vi "ClassProvidor_GoopOptionsDialog.vi"(8 "error in (no error)":errorcluster) -> (0 "error out":errorcluster)   [LabVIEW 2020]
uses:
  Provider_EndevoGOOP300/EndevoProviderName.ctl
  Provider_EndevoGOOP400/EndevoG4ProviderName.ctl
panel:
  out "ProductPicture":picture
  in  "_InstallNewClassProvider":bool
  in  "_RemoveClassProvider":bool
  in  "_HelpGoopOption":bool
  in  "_AddClassProvider":bool
  out "Tab":enum32{"Select", "Add"}(tab)
  in  "ModifyProviders":bool
  in  "_CurrentClassProvider":u16(ring) caption="Current Class provider to use:" items=["LVClass by value", "By Reference (GOOP3)", "By Reference DVR (GOOP4)"]
  in  "_ConfigureCurrentClassProvider":bool
  in  "_ProviderClassReaderPath":path caption="Provider Class Reader Path"
  in  "_ProviderClassWriterPath":path caption="Provider Class Writer Path"
  in  "_ProviderName":string caption="ProviderName"
  in  "Cancel":bool
  in  "OK":bool
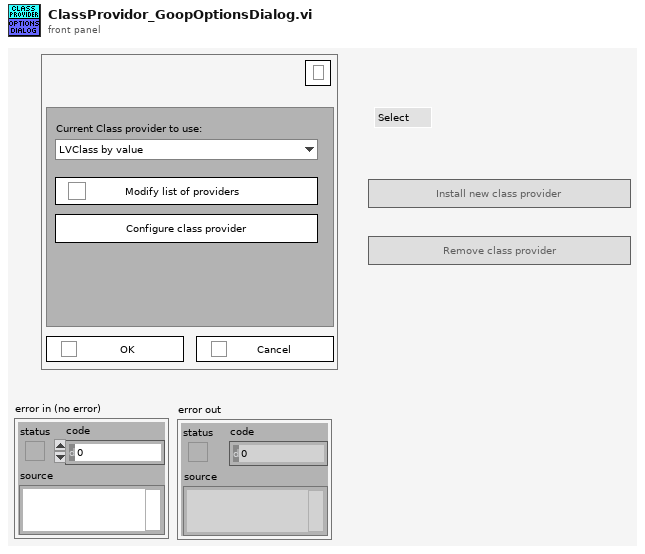
[diagram p1: front panel]
types:
  T1 = cluster{"ClassProviders":string[], "Path":path, "ClassConfig":path, "ClassProviders(Translated)":string[]}
  T2 = typedef "EndevoG4ProviderName.ctl" = enum16{"EndevoGOOP400"}
  T3 = typedef "EndevoProviderName.ctl" = enum16{"EndevoGOOP300"}
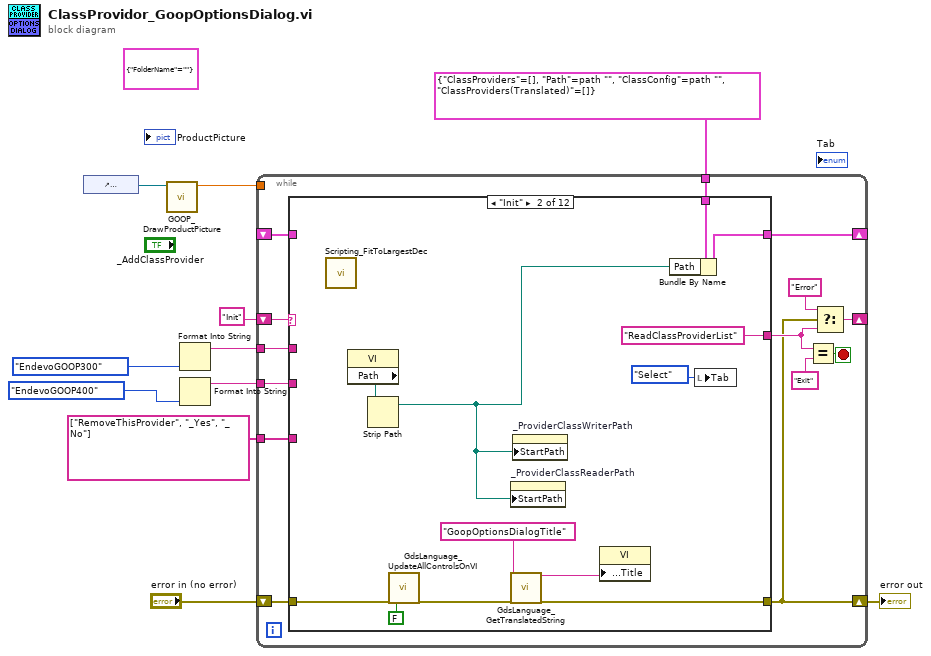
[diagram p0: block diagram]
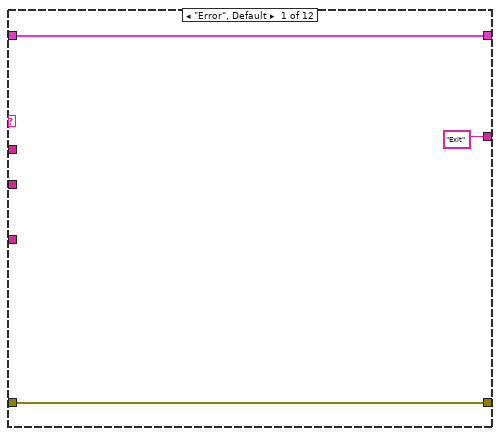
[diagram p2: hidden frame]
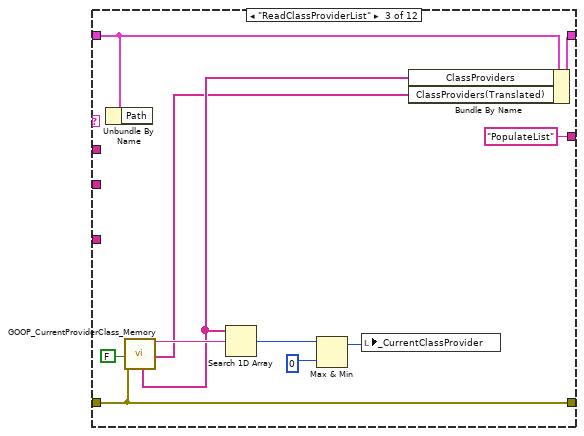
[diagram p3: hidden frame]
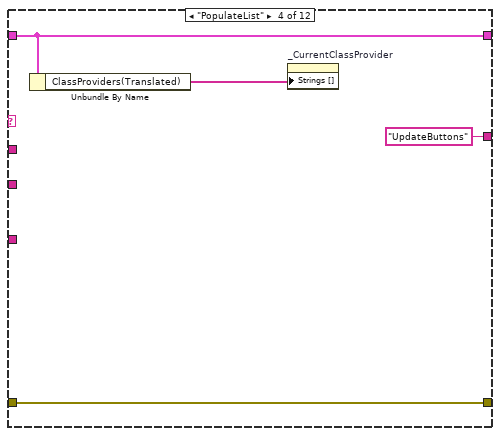
[diagram p4: hidden frame]
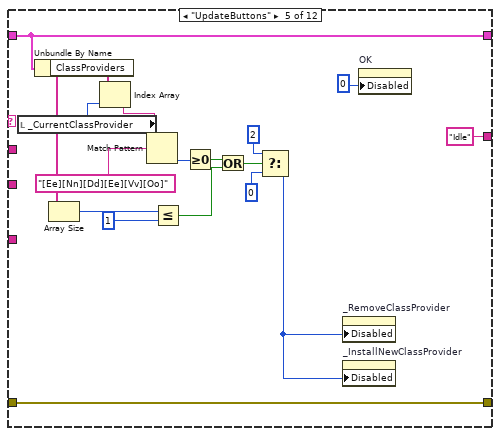
[diagram p5: hidden frame]
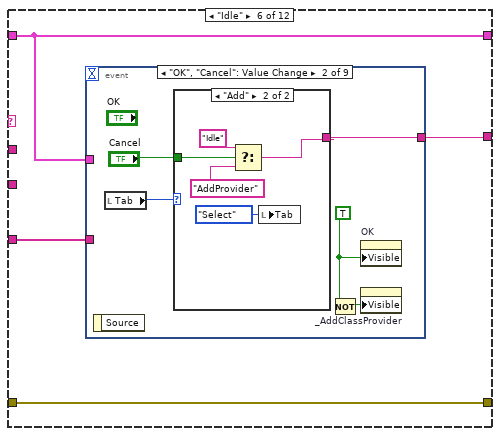
[diagram p6: hidden frame]
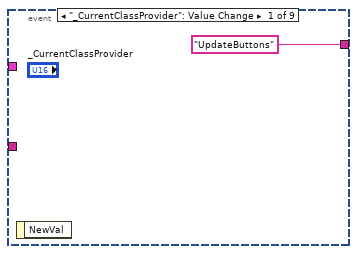
[diagram p7: hidden frame]
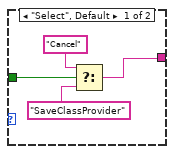
[diagram p8: hidden frame]
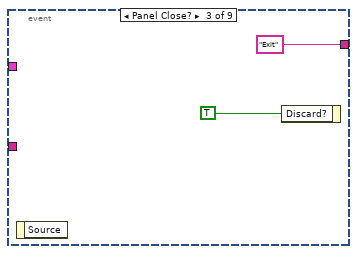
[diagram p9: hidden frame]
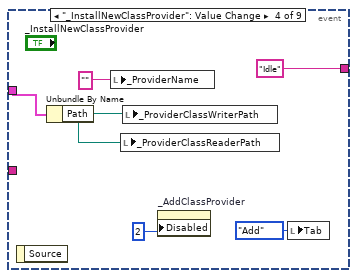
[diagram p10: hidden frame]
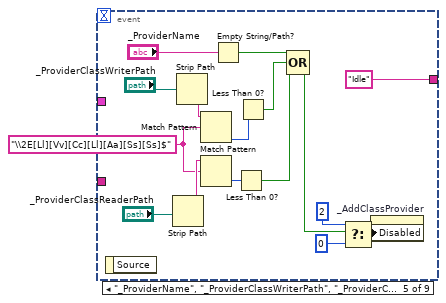
[diagram p11: hidden frame]
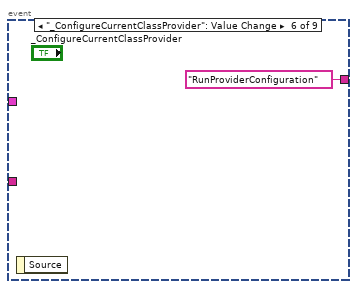
[diagram p12: hidden frame]
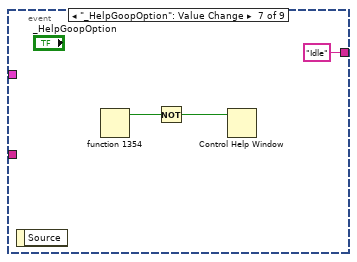
[diagram p13: hidden frame]
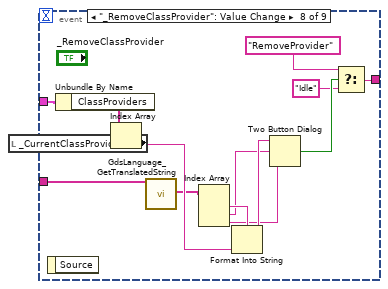
[diagram p14: hidden frame]
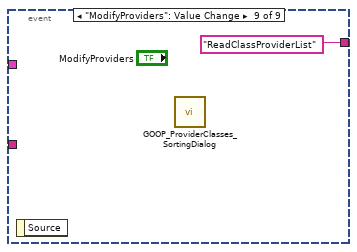
[diagram p15: hidden frame]
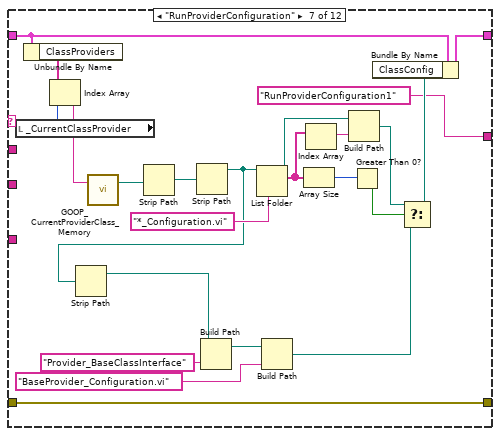
[diagram p16: hidden frame]
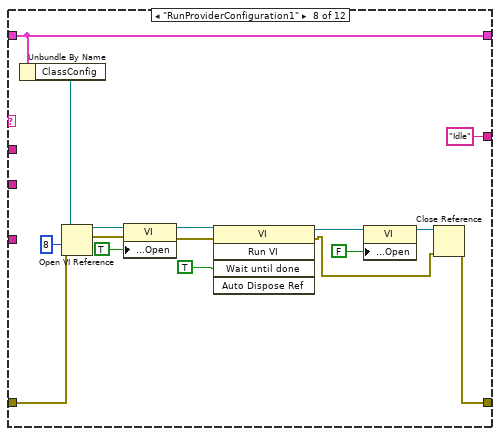
[diagram p17: hidden frame]
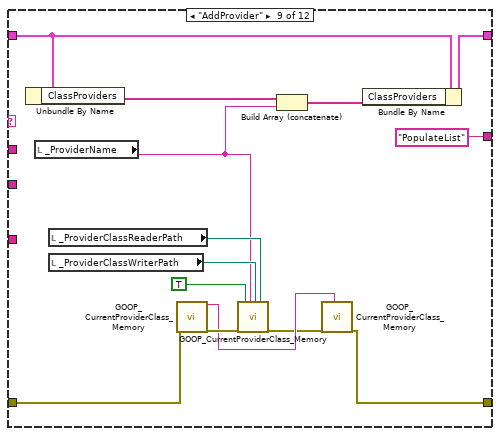
[diagram p18: hidden frame]
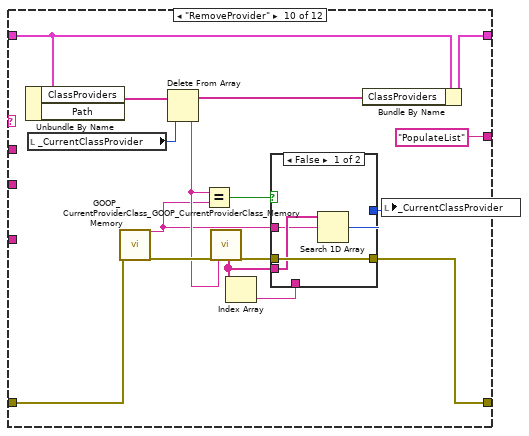
[diagram p19: hidden frame]
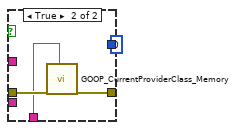
[diagram p20: hidden frame]
diagram:
  (unwired) cluster{"FolderName":string} {"FolderName"=""}
  n1 = control-ref of="ProductPicture"() -> (w3:refnum<vi>)
  n2 = call "GOOP_DrawProductPicture.vi"("ProductPictureControl"=w3) -> ("Zoom Factor"=w2:sgl)  [unwired: 10 in]
  n3 = Format Into String(EndevoProviderName."EndevoGOOP300" ("ProviderName")) -> (resulting string=w5:string)  [unwired: 3 in, 1 out]
  n4 = Format Into String(EndevoG4ProviderName."EndevoGOOP400" ("ProviderName")) -> (resulting string=w4:string)  [unwired: 3 in, 1 out]
  n5 = while {
    shift-right: [w18] -> w9
    shift-left: "error in (no error)" -> [w25]
    shift-right: [w23] -> _
    shift-left: "Init" -> [w24]
    shift-right: [w17] -> _
    shift-left: _ -> [w16]
    tunnel: string[] ["RemoveThisProvider", "_Yes", "_No"] -> [w15]
    tunnel: w5 -> [w14]
    tunnel: w4 -> [w13]
    tunnel: w2 -> [_]
    tunnel: T1 {"ClassProviders"=[], "Path"=path "", "ClassConfig"=path "", "ClassProviders(Translated)"=[]} -> [w12]
    stop <- w22 stop-if-true
    n6 = case shown="\"Init\"" w24 {
      tunnel: w25 -> [w28 w34 w49 w53 w60 w75 w154 w172 w178 w197 w216 w219]
      tunnel: [w28 w31 w49 w53 w60 w75 w154 w170 w174 w191 w215 w219] -> w18
      tunnel: ["Exit" "ReadClassProviderList" "PopulateList" "UpdateButtons" "Idle" w76 "RunProviderConfiguration1" "Idle" ("f") "PopulateList" "PopulateList" "Exit" "Exit"] -> w19
      tunnel: [w26 w38 w50 w54 w62 w74 w152 w169 w187 w203 w218 w221] -> w17
      tunnel: w16 -> [w26 _ w46 w54 w62 w74 w153 w169 w186 w202 w218 w221]
      tunnel: w15 -> [_ _ _ _ _ w73 _ _ _ _ _ _]
      tunnel: w14 -> [_ _ _ _ _ _ _ _ _ _ _ _]
      tunnel: w13 -> [_ _ _ _ _ _ _ _ _ _ _ _]
      tunnel: w12 -> [_ w29 _ _ _ _ _ _ _ _ _ _]
      frame "Error", Default {
      }
      frame "Init" {
        n7 = call "Scripting_FitToLargestDec.vi"() -> ()  [unwired: 6 in, 2 out]
        n8 = property class="VI"() -> ("Path"=w37:path)  [unwired: 2 in, 2 out]
        n9 = Strip Path(path=w37) -> (stripped path=w36:path)  [unwired: 1 out]
        n10 = call "GdsLanguage_UpdateAllControlsOnVI.vi"("error in (no error)"=w34, "CreateLanguageFile(Use this to create a languageFile)"=FALSE) -> ("error out"=w33:errorcluster)  [unwired: 16 in, 1 out]
        n11 = property on="_ProviderClassReaderPath" class="Path"("StartPath"=w36) -> ()  [unwired: 2 in, 2 out]
        n12 = call "GdsLanguage_GetTranslatedString.vi"("StringID(s)"="GoopOptionsDialogTitle", "error in (no error)"=w33) -> ("FirstStringOut"=w30:string, "error out"=w31:errorcluster)  [unwired: 14 in, 2 out]
        n13 = property on="_ProviderClassWriterPath" class="Path"("StartPath"=w36) -> ()  [unwired: 2 in, 2 out]
        n14 = property class="VI"("Front Panel.Title"=w30) -> ()  [unwired: 2 in, 2 out]
        n15 = Bundle By Name(cluster=w29, "Path"=w36) -> (w38:T1)
        n16 = local write "Tab"(enum32{"Select", "Add"}."Select" ("Tab")) -> ()
      }
      frame "ReadClassProviderList" {
        n17 = Unbundle By Name(w46) -> ()  [unwired: 1 out]
        n18 = call "GOOP_CurrentProviderClass_Memory.vi"("IgnoreFilter(False)"=FALSE, "error in (no error)"=w49) -> ("AllClassProviders(OriginalNames)"=w47:string[], "ClassProviderName"=w48:string, "AllClassProviders(TranslatedNames)"=w42:string[])  [unwired: 11 in, 4 out]
        n19 = Search 1D Array(1D array=w47, element=w48) -> (index of element=w45:i32)  [unwired: 1 in]
        n20 = Max & Min(x=w45, y=0 ("lower limit")) -> (max(x,y)=w43:i32)  [unwired: 1 out]
        n21 = local write "_CurrentClassProvider"(w43) -> ()
        n22 = Bundle By Name(cluster=w46, "ClassProviders"=w47, "ClassProviders(Translated)"=w42) -> (w50:T1)
      }
      frame "PopulateList" {
        n23 = Unbundle By Name(w54) -> ("ClassProviders(Translated)"=w52:string[])
        n24 = property on="_CurrentClassProvider" class="Ring (strict)"("Strings []"=w52) -> ()  [unwired: 2 in, 2 out]
      }
      frame "UpdateButtons" {
        n25 = local read "_CurrentClassProvider"() -> (w58:u16)
        n26 = Unbundle By Name(w62) -> ("ClassProviders"=w71:string[])
        n27 = Array Size(array=w71) -> (size(s)=w69:i32)
        n28 = Index Array(array=w71, index=w58) -> (element=w57:string)
        n29 = Match Pattern(string=w57, regular expression="[Ee][Nn][Dd][Ee][Vv][Oo]") -> (offset past match=w70:i32)  [unwired: 1 in, 3 out]
        n30 = Less Or Equal?(x=w69, y=1) -> (x <= y?=w66:bool)
        n31 = Greater Or Equal To 0?(x=w70) -> (x >= 0?=w67:bool)
        n32 = Or(x=w67, y=w66) -> (x .or. y?=w65:bool)
        n33 = Select(t=u8 2 ("Disabled"), s=w65, f=u8 0 ("Disabled")) -> (s? t:f=w56:u8)
        n34 = property on="_RemoveClassProvider" class="Bool"("Disabled"=w56) -> ()  [unwired: 2 in, 2 out]
        n35 = property on="_InstallNewClassProvider" class="Bool"("Disabled"=w56) -> ()  [unwired: 2 in, 2 out]
        n36 = property on="OK" class="Bool"("Disabled"=u8 0) -> ()  [unwired: 2 in, 2 out]
      }
      frame "Idle" {
        n37 = event shown="[1] \"OK\", \"Cancel\": Value Change" {
          selector: _ -> [_ _ _ _ _ _ _ _ _]
          dyn-events: _ -> [_ _ _ _ _ _ _ _ _]
          timeout: _ -> [_ _ _ _ _ _ _ _ _]
          tunnel: ["UpdateButtons" w80 "Exit" "Idle" "Idle" "RunProviderConfiguration" ("f") "Idle" ("f") w127 "ReadClassProviderList"] -> w76
          tunnel: w74 -> [_ _ _ w95 _ _ _ w133 _]
          tunnel: w73 -> [_ _ _ _ _ _ _ w122 _]
          event "_CurrentClassProvider": Value Change {
            n38 = event-data() -> ()  [unwired: 1 in, 1 out]
          }
          event "OK", "Cancel": Value Change {
            w78 = TRUE ("Visible")
            n39 = event-data() -> ()  [unwired: 1 in, 1 out]
            n40 = local read "Tab"() -> (w82:enum32{"Select", "Add"})
            n41 = case shown="\"Add\"" w82 {
              tunnel: "Cancel" -> [w86 w91]
              tunnel: [w85 w88] -> w80
              frame "Select", Default {
                n42 = Select(t="Cancel", s=w86, f="SaveClassProvider") -> (s? t:f=w85:string)
              }
              frame "Add" {
                n43 = Select(t="Idle", s=w91, f="AddProvider") -> (s? t:f=w88:string)
                n44 = local write "Tab"(enum32{"Select", "Add"}."Select" ("Tab")) -> ()
              }
            }
            n45 = Not(x=w78) -> (.not. x?=w79:bool)
            n46 = property on="OK" class="Bool"("Visible"=w78) -> ()  [unwired: 2 in, 2 out]
            n47 = property on="_AddClassProvider" class="Bool"("Visible"=w79) -> ()  [unwired: 2 in, 2 out]
          }
          event Panel Close? {
            n48 = event-data() -> ()  [unwired: 1 in, 1 out]
            n49 = event-data("Discard?"=TRUE) -> ()  [unwired: 1 in, 1 out]
          }
          event "_InstallNewClassProvider": Value Change {
            n50 = event-data() -> ()  [unwired: 1 in, 1 out]
            n51 = Unbundle By Name(w95) -> ("Path"=w94:path)
            n52 = local write "_ProviderName"("" ("Provider folder name:")) -> ()
            n53 = local write "_ProviderClassReaderPath"(w94) -> ()
            n54 = local write "_ProviderClassWriterPath"(w94) -> ()
            n55 = property on="_AddClassProvider" class="Bool"("Disabled"=u8 2) -> ()  [unwired: 2 in, 2 out]
            n56 = local write "Tab"(enum32{"Select", "Add"}."Add" ("Tab")) -> ()
          }
          event "_ProviderName", "_ProviderClassWriterPath", "_ProviderClassReaderPath": Value Change {
            w102 = "\\2E[Ll][Vv][Cc][Ll][Aa][Ss][Ss]$" ("regular expression")
            n57 = event-data() -> ()  [unwired: 1 in, 1 out]
            n58 = Strip Path(path="_ProviderClassReaderPath") -> (name=w103:string)  [unwired: 1 out]
            n59 = Strip Path(path="_ProviderClassWriterPath") -> (name=w107:string)  [unwired: 1 out]
            n60 = Match Pattern(string=w107, regular expression=w102) -> (offset past match=w106:i32)  [unwired: 1 in, 3 out]
            n61 = Match Pattern(string=w103, regular expression=w102) -> (offset past match=w101:i32)  [unwired: 1 in, 3 out]
            n62 = Empty String/Path?(string/path="_ProviderName") -> (empty?=w110:bool)
            n63 = Less Than 0?(x=w101) -> (x < 0?=w100:bool)
            n64 = Less Than 0?(x=w106) -> (x < 0?=w105:bool)
            n65 = Compound Arithmetic op=OR(w110, w105, w100) -> (w109:bool)
            n66 = Select(t=u8 2 ("Disabled"), s=w109, f=u8 0) -> (s? t:f=w113:u8)
            n67 = property on="_AddClassProvider" class="Bool"("Disabled"=w113) -> ()  [unwired: 2 in, 2 out]
          }
          event "_ConfigureCurrentClassProvider": Value Change {
            n68 = event-data() -> ()  [unwired: 1 in, 1 out]
          }
          event "_HelpGoopOption": Value Change {
            n69 = event-data() -> ()  [unwired: 1 in, 1 out]
            n70 = fn#1354() -> (1:w119:bool)  [unwired: 1 out]
            n71 = Not(x=w119) -> (.not. x?=w118:bool)
            n72 = Control Help Window(1:w118) -> ()  [unwired: 1 in]
          }
          event "_RemoveClassProvider": Value Change {
            n73 = local read "_CurrentClassProvider"() -> (w131:u16)
            n74 = event-data() -> ()  [unwired: 1 in, 1 out]
            n75 = Unbundle By Name(w133) -> ("ClassProviders"=w132:string[])
            n76 = Index Array(array=w132, index=w131) -> (element=w125:string)
            n77 = call "GdsLanguage_GetTranslatedString.vi"("StringID(s)"=w122) -> ("StringsOut"=w124:string[])  [unwired: 15 in, 3 out]
            n78 = Index Array(array=w124) -> (element #1=w123:string, element #2=w121:string, element #3=w120:string)  [unwired: 3 in]
            n79 = Format Into String(format string=w123, w125) -> (resulting string=w130:string)  [unwired: 2 in, 1 out]
            n80 = Two Button Dialog(message=w130, 1:w120, 2:w121) -> (T button?=w129:bool)
            n81 = Select(t="RemoveProvider", s=w129, f="Idle") -> (s? t:f=w127:string)
          }
          event "ModifyProviders": Value Change {
            n82 = event-data() -> ()  [unwired: 1 in, 1 out]
            n83 = call "GOOP_ProviderClasses_SortingDialog.vi"() -> ()  [unwired: 9 in, 3 out]
          }
        }
      }
      frame "RunProviderConfiguration" {
        n84 = local read "_CurrentClassProvider"() -> (w156:u16)
        n85 = Unbundle By Name(w153) -> ("ClassProviders"=w157:string[])
        n86 = Index Array(array=w157, index=w156) -> (element=w155:string)
        n87 = call "GOOP_CurrentProviderClass_Memory.vi"("GetThisClassProvidersPaths(Returns the default providor if not wired)"=w155) -> ("ClassProviderClassWriterPath"=w146:path)  [unwired: 12 in, 6 out]
        n88 = Strip Path(path=w146) -> (stripped path=w145:path)  [unwired: 1 out]
        n89 = Strip Path(path=w145) -> (stripped path=w136:path)  [unwired: 1 out]
        n90 = Strip Path(path=w136) -> (stripped path=w135:path)  [unwired: 1 out]
        n91 = Build Path(base path=w135, name or relative path="Provider_BaseClassInterface") -> (appended path=w148:path)
        n92 = List Folder(path=w136, pattern="*_Configuration.vi" ("name or relative path")) -> (path out=w138:path, filenames=w140:string[])  [unwired: 2 in, 2 out]
        n93 = Build Path(base path=w148, name or relative path="BaseProvider_Configuration.vi") -> (appended path=w142:path)
        n94 = Array Size(array=w140) -> (size(s)=w143:i32)
        n95 = Index Array(array=w140) -> (element=w139:string)  [unwired: 1 in]
        n96 = Build Path(base path=w138, name or relative path=w139) -> (appended path=w137:path)
        n97 = Greater Than 0?(x=w143) -> (x > 0?=w141:bool)
        n98 = Select(t=w137, s=w141, f=w142) -> (s? t:f=w151:path)
        n99 = Bundle By Name(cluster=w153, "ClassConfig"=w151) -> (w152:T1)
      }
      frame "RunProviderConfiguration1" {
        n100 = Unbundle By Name(w169) -> ("ClassConfig"=w173:path)
        n101 = Open VI Reference(vi path=w173, options=8, error in (no error)=w172) -> (vi reference=w166:refnum<vi>, error out=w167:errorcluster)  [unwired: 3 in]
        n102 = property class="VI"(reference=w166, error in=w167, "Front Panel.Open"=TRUE ("Front Panel Window:Open")) -> (reference out=w165:refnum<vi>, error out=w164:errorcluster)
        n103 = invoke class="VI" method="Run VI"(reference=w165, error in=w164, "Wait until done"=TRUE ("Wait Until Done")) -> (reference out=w161:refnum<vi>, error out=w159:errorcluster)  [unwired: 2 in, 3 out]
        n104 = property class="VI"(reference=w161, "Front Panel.Open"=FALSE ("Front Panel Window:Open")) -> (reference out=w160:refnum<vi>)  [unwired: 1 in, 1 out]
        n105 = Close Reference(reference=w160, error in (no error)=w159) -> (error out=w170:errorcluster)
      }
      frame "AddProvider" {
        n106 = Unbundle By Name(w186) -> ("ClassProviders"=w185:string[])
        n107 = local read "_ProviderName"() -> (w180:string)
        n108 = local read "_ProviderClassReaderPath"() -> (w181:path)
        n109 = local read "_ProviderClassWriterPath"() -> (w182:path)
        n110 = call "GOOP_CurrentProviderClass_Memory.vi"("error in (no error)"=w178) -> ("ClassProviderName"=w176:string, "error out"=w177:errorcluster)  [unwired: 12 in, 5 out]
        n111 = call "GOOP_CurrentProviderClass_Memory.vi"("error in (no error)"=w177, "Don't Set just update"=TRUE, "SetDefaultClassProvider(Ignored if not wired)"=w180, "ClassProviderClassWriterPath(Used if not empty)"=w182, "ClassProviderClassReaderPath(Used if not empty)"=w181) -> ("error out"=w175:errorcluster)  [unwired: 8 in, 6 out]
        n112 = Build Array (concatenate)(w185, w180) -> (w184:string[])
        n113 = call "GOOP_CurrentProviderClass_Memory.vi"("error in (no error)"=w175, "SetDefaultClassProvider(Ignored if not wired)"=w176) -> ("error out"=w174:errorcluster)  [unwired: 11 in, 6 out]
        n114 = Bundle By Name(cluster=w186, "ClassProviders"=w184) -> (w187:T1)
      }
      frame "RemoveProvider" {
        n115 = Unbundle By Name(w202) -> ("ClassProviders"=w200:string[])  [unwired: 1 out]
        n116 = local read "_CurrentClassProvider"() -> (w198:u16)
        n117 = call "GOOP_CurrentProviderClass_Memory.vi"("error in (no error)"=w197) -> ("ClassProviderName"=w188:string, "error out"=w196:errorcluster)  [unwired: 12 in, 5 out]
        n118 = Delete From Array(array=w200, index=w198) -> (deleted portion=w195:string, array with subset deleted=w199:string[])  [unwired: 1 in]
        n119 = Equal?(x=w195, y=w188) -> (x = y?=w194:bool)
        n120 = call "GOOP_CurrentProviderClass_Memory.vi"("error in (no error)"=w196, "RemoveThisClassProvidersPaths(Ignored if not wired)"=w195) -> ("AllClassProviders(OriginalNames)"=w189:string[], "error out"=w193:errorcluster)  [unwired: 11 in, 5 out]
        n121 = Index Array(array=w189) -> (element=w192:string)  [unwired: 1 in]
        n122 = case shown="False" w194 {
          tunnel: w193 -> [w207 w211]
          tunnel: w192 -> [_ w210]
          tunnel: [w207 w209] -> w191
          tunnel: [w204 u16 0 ("x")] -> w190
          tunnel: w189 -> [w206 _]
          tunnel: w188 -> [w205 _]
          frame False {
            n123 = Search 1D Array(1D array=w206, element=w205) -> (index of element=w204:i32)  [unwired: 1 in]
          }
          frame True {
            n124 = call "GOOP_CurrentProviderClass_Memory.vi"("error in (no error)"=w211, "SetDefaultClassProvider(Ignored if not wired)"=w210) -> ("error out"=w209:errorcluster)  [unwired: 11 in, 6 out]
          }
        }
        n125 = Bundle By Name(cluster=w202, "ClassProviders"=w199) -> (w203:T1)
        n126 = local write "_CurrentClassProvider"(w190) -> ()
      }
      frame "SaveClassProvider" {
        n127 = Unbundle By Name(w218) -> ("ClassProviders"=w214:string[])
        n128 = local read "_CurrentClassProvider"() -> (w213:u16)
        n129 = Index Array(array=w214, index=w213) -> (element=w212:string)
        n130 = call "GOOP_CurrentProviderClass_Memory.vi"("error in (no error)"=w216, "SetDefaultClassProvider(Ignored if not wired)"=w212) -> ("error out"=w215:errorcluster)  [unwired: 11 in, 6 out]
      }
      frame "Cancel" {
      }
    }
    n131 = Equal?(x=w19, y="Exit") -> (x = y?=w22:bool)
    n132 = Select(t="Error", s=w18, f=w19) -> (s? t:f=w23:string)
  }
  "error out" <- w9
